vi "RemoteVI Serve Pending Connection.vi"(0 "pending":T1, 1 "token":string, 5 "html":string, 7 "max clients reached?":bool, 9 "now":u32) -> (4 "pending out":T1, 6 "keep?":bool, 8 "websocket?":bool)   [LabVIEW 2020, in "RemoteVI.lvlib"]
doc: "One step for one pending (accepted but not yet answered) connection, without blocking: reads what has arrived of the request head (RemoteVI Read Request Head.vi, timeout 0). A complete head is served by RemoteVI Handle Connection.vi (keep? FALSE; websocket? TRUE when it was upgraded - the caller then owns the connection as a client). A connection that is gone or has been pending for 5 s or more (now - accepted, a browser's speculative preconnect that never sends a request) is closed (keep? FALSE). Otherwise it stays pending with the bytes read so far (keep? TRUE). connection is the TCP connection refnum type-cast to U32."
uses:
  RemoteVI.lvlib
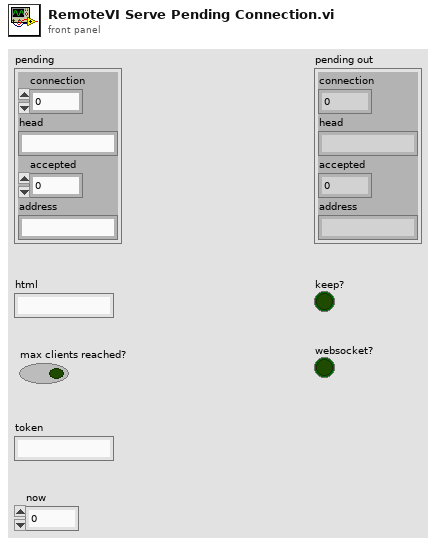
[diagram p1: front panel]
types:
  T1 = cluster{"connection":u32, "head":string, "accepted":u32, "address":string}
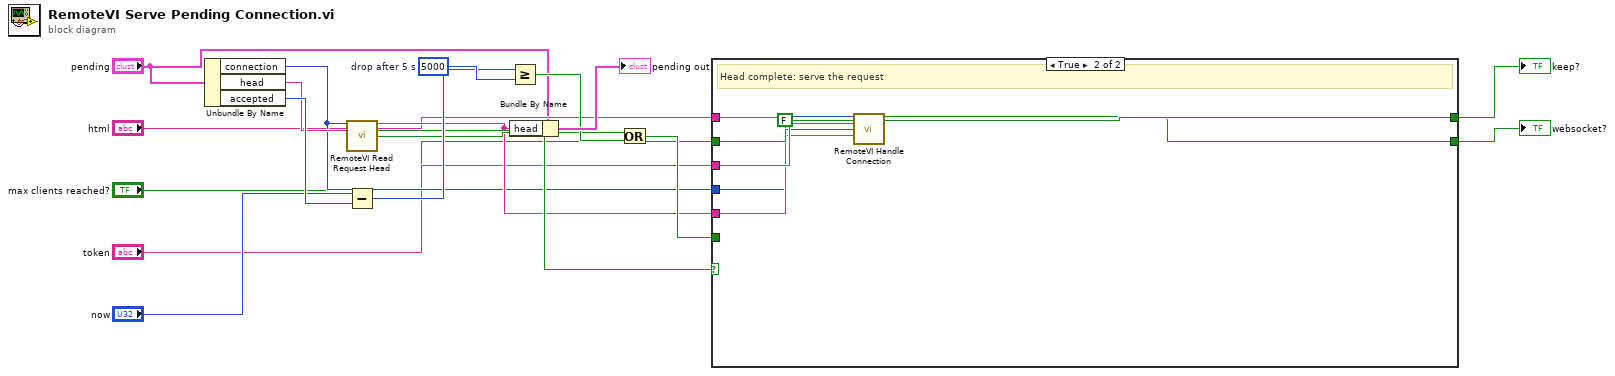
[diagram p0: block diagram]
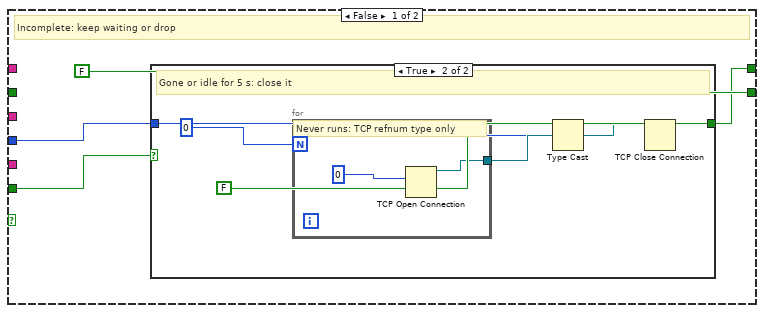
[diagram p2: hidden frame]
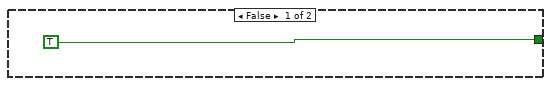
[diagram p3: hidden frame]
diagram:
  w13 = u32 5000  # drop after 5 s
  n1 = Unbundle By Name("pending") -> ("connection"=w6:u32, "head"=w7:string, "accepted"=w8:u32)
  n2 = call "RemoteVI Read Request Head.vi"("connection"=w6, "head in"=w7) -> ("head out"=w9:string, "complete?"=w10:bool, "gone?"=w11:bool)  [unwired: 11 in]
  n3 = Subtract(x="now", y=w8) -> (x-y=w12:u32)
  n4 = Greater Or Equal?(x=w12, y=w13) -> (x >= y?=w14:bool)
  n5 = Bundle By Name(cluster="pending", "head"=w9) -> (→"pending out":T1)
  n6 = Or(x=w11, y=w14) -> (x .or. y?=w15:bool)
  n7 = case shown="True" w10 {
    tunnel: "html" -> [_ w33]
    tunnel: "max clients reached?" -> [_ w34]
    tunnel: "token" -> [_ w35]
    tunnel: [w21 FALSE] -> w17
    tunnel: w6 -> [w19 w31]
    tunnel: w9 -> [_ w32]
    tunnel: w15 -> [w20 _]
    tunnel: [FALSE w36] -> w18
    frame False {
      # "Incomplete: keep waiting or drop"
      n8 = case shown="True" w20 {
        tunnel: [TRUE FALSE] -> w21
        tunnel: w19 -> [_ w24]
        frame False {
        }
        frame True {
          # "Gone or idle for 5 s: close it"
          n9 = for {
            N: 0 -> [_]
            tunnel: [w30] -> w26
            # "Never runs: TCP refnum type only"
            n10 = TCP Open Connection(remote port or service name=u16 0) -> (connection ID=w30:refnum<k5>)  [unwired: 4 in, 1 out]
          }
          n11 = Type Cast(type=w26, x=w24) -> (*(type *) &x=w27:refnum<k5>)
          n12 = TCP Close Connection(connection ID=w27) -> ()  [unwired: 2 in, 2 out]
        }
      }
    }
    frame True {
      # "Head complete: serve the request"
      n13 = call "RemoteVI Handle Connection.vi"("connection"=w31, "token"=w35, "html"=w33, "max clients reached?"=w34, "request head"=w32) -> ("websocket?"=w36:bool)  [unwired: 9 in, 1 out]
    }
  }
  "keep?" <- w17
  "websocket?" <- w18
